vi "FileDialogWithEvent.vi"(0 "start path":path=path "", 1 "default name":string, 2 "File dialog event":T1, 5 "pattern (all files)":string, 7 "pattern label":string, 9 "selection mode":T3(ring)=enum."new or existing file", 11 "error in":errorcluster, 12 "prompt":string, 13 "button label":string) -> (4 "selected paths":path[](array[path]), 15 "error out":errorcluster)   [LabVIEW 2025]
uses:
  FileDialogResult.ctl
  FileDialogEvent.ctl
panel:
  in  "File dialog result":T2
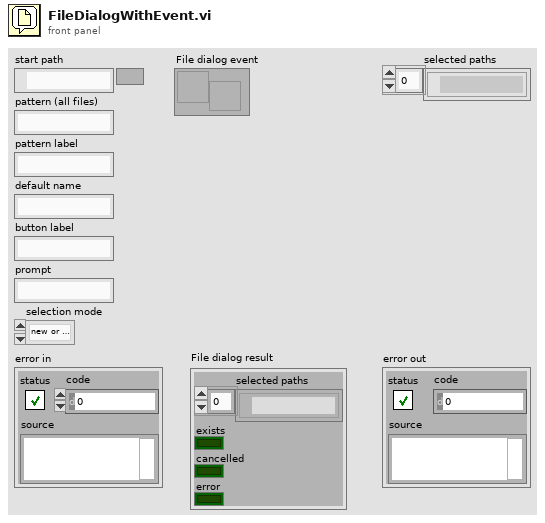
[diagram p1: front panel]
types:
  T1 = typedef "FileDialogEvent.ctl" = refnum<user-event>
  T2 = typedef "FileDialogResult.ctl" = cluster{"selected paths":path[], "exists":bool, "cancelled":bool, "error":bool}
  T3 = enum32{"existing file", "new file", "new or existing file", "existing dir", "new dir", "new or existing dir", "existing file (use LLBs)", "new file (use LLBs)", "new or existing file (use LLBs)", "new or existing file or directory (use LLBs)", "existing dir (use LLBs)", "new dir (use LLBs)", "new or existing dir (use LLBs)", "existing file or dir", "new file or dir", "new or existing file or dir", "existing file or dir (use LLBs)", "new file or dir (use LLBs)", "multi-select", "multi-select (use LLBs)"}
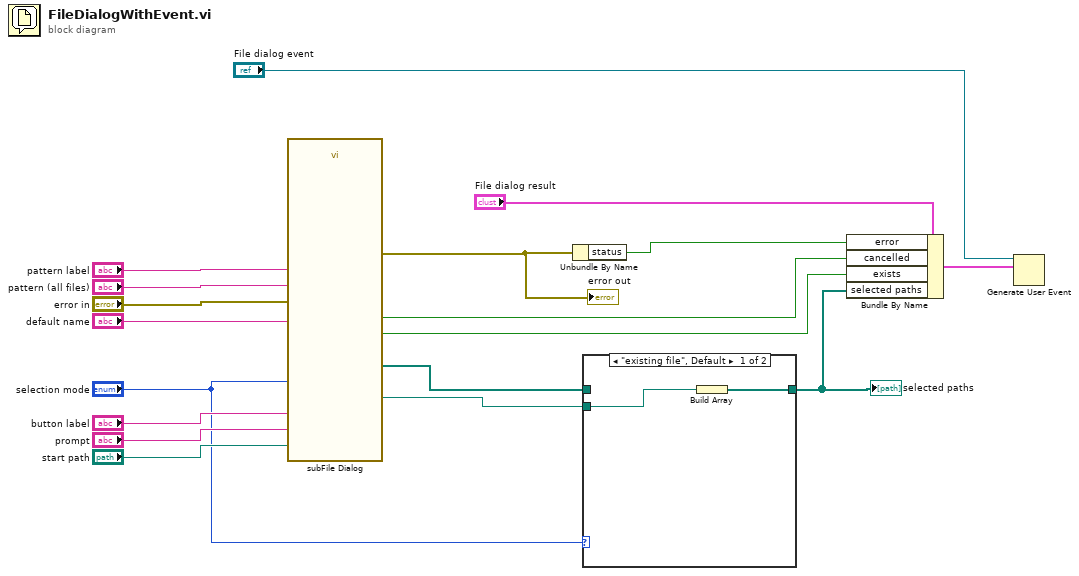
[diagram p0: block diagram]
diagram:
  n1 = call <vilib>:"subFile Dialog.vi"("start path"="start path", "prompt"="prompt", "button label"="button label", "selection mode"="selection mode", "default name"="default name", "error in"="error in", "pattern (all files)"="pattern (all files)", "pattern label"="pattern label") -> ("selected path"=w9:path, "selected paths"=w10:path[], "exists"=w4:bool, "cancelled"=w5:bool, "error out"=w7:errorcluster)  [unwired: 3 in]
  "error out" <- w7
  n2 = Unbundle By Name(w7) -> ("status"=w6:bool)
  n3 = case shown="\"existing file\", Default" "selection mode" {
    tunnel: w10 -> [_ w21]
    tunnel: w9 -> [w19 _]
    tunnel: [w20 w21] -> w1
    frame "existing file", Default {
      n4 = Build Array(w19) -> (w20:path[])
    }
    frame "multi-select", "multi-select (use LLBs)" {
    }
  }
  "selected paths" <- w1
  n5 = Bundle By Name(cluster="File dialog result", "error"=w6, "cancelled"=w5, "exists"=w4, "selected paths"=w1) -> (w2:T2)
  n6 = Generate User Event(user event="File dialog event", event data cluster=w2) -> ()  [unwired: 2 in, 2 out]
